vi "Debug Line.vi"(11 "UIMessage in":refnum<class "UIMessage.lvclass">) -> (2 "Debug Line":string, 3 "UIMessage out":refnum<class "UIMessage.lvclass">)   [LabVIEW 2020, in "TSnax.lvlib" / "UIMessage.lvclass"]
uses:
  UIMessage.lvclass
  UIMessage.lvclass/UIMessage.ctl
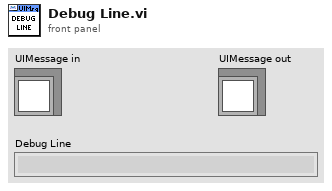
[diagram p1: front panel]
types:
  T1 = typedef "TSnax.lvlib/UIMsg.ctl" = enum16{"Unknown", "BreakOnUserRequest", "BreakOnBreakpoint", "BreakOnRunTimeError", "Trace", "TerminatingExecution", "AbortingExecution", "KillingExecutionThreads", "EndExecution", "ShutDownComplete", "StartExecution", "ProgressPercent", "ProgressText", "StartInteractiveExecution", "EndInteractiveExecution", "TerminatingInteractiveExecution", "TerminationCancelled", "ResumeFromBreak", "StartFileExecution", "EndFileExecution", "ShutDownCancelled", "LocalizationSettingChanged", "OpenWindows", "TileWindows", "CascadeWindows", "ReportChanged", "CloseWindows", "RefreshWindows", "ClientFileChanged", "DisplayReport", "ModelState_Initializing", "ModelState_Waiting", "ModelState_Identified", "ModelState_BeginTesting", "ModelState_TestingComplete", "ModelState_PostProcessingComplete", "ModelState_EnabledStateSet", "ReportLocationChanged", "GotoLocation", "PushUndoItem", "OutputMessages", "TypePaletteFileListChanged", "NonTerminatingThreadsArePreventingTermination", "ModelState_PostProcessing", "ReportCollectionChanged", "RuntimeError"}
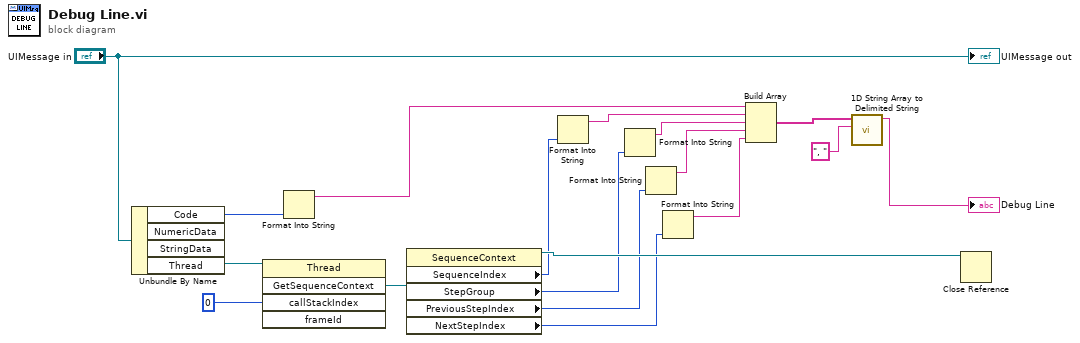
[diagram p0: block diagram]
diagram:
  n1 = Unbundle By Name("UIMessage in") -> ("Code"=w13:T1, "Thread"=w14:refnum<k7>)  [unwired: 2 out]
  n2 = invoke class="Thread" method="GetSequenceContext"(reference=w14, "callStackIndex"=0) -> ("GetSequenceContext"=w16:refnum<k7>)  [unwired: 3 in, 4 out]
  n3 = Format Into String(w13) -> (resulting string=w11:string)  [unwired: 3 in, 1 out]
  n4 = property class="SequenceContext"(reference=w16) -> (reference out=w15:refnum<k7>, "SequenceIndex"=w12:i32, "StepGroup"=w9:i32, "PreviousStepIndex"=w7:i32, "NextStepIndex"=w2:i32)  [unwired: 1 in, 1 out]
  n5 = Format Into String(w12) -> (resulting string=w10:string)  [unwired: 3 in, 1 out]
  n6 = Format Into String(w9) -> (resulting string=w8:string)  [unwired: 3 in, 1 out]
  n7 = Format Into String(w7) -> (resulting string=w6:string)  [unwired: 3 in, 1 out]
  n8 = Format Into String(w2) -> (resulting string=w1:string)  [unwired: 3 in, 1 out]
  n9 = Build Array(w11, w10, w8, w6, w1) -> (w5:string[])
  n10 = call <vilib>:"1D String Array to Delimited String.vi"("delimiter"=", ", "string array"=w5) -> ("delimited string"=→"Debug Line":string)  [unwired: 9 in]
  n11 = Close Reference(reference=w15) -> ()  [unwired: 1 in, 1 out]
  "UIMessage out" <- "UIMessage in"
